vi "FlatToRichcif_can_writer_nixnet_GetCANStatusResponse.vi"(5 "OutputClusterType":T1, 11 "InputCluster":T4) -> (3 "OutputCluster":T1)   [LabVIEW 2021, in "CanWriterNixnet_client.lvlib"]
uses:
  CanWriterNixnet_client.lvlib
  cif_can_writer_nixnet_GetCANStatusResponse_Flat.ctl
  cif_can_writer_nixnet_CommState.ctl
  cif_can_writer_nixnet_LastError.ctl
  cif_can_writer_nixnet_GetCANStatusResponse.ctl
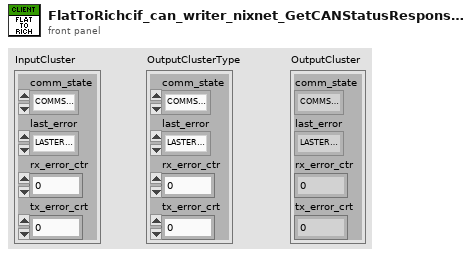
[diagram p1: front panel]
types:
  T1 = typedef "CanWriterNixnet_client.lvlib/cif_can_writer_nixnet_GetCANStatusResponse.ctl" = cluster{"comm_state":T2, "last_error":T3, "rx_error_ctr":u32, "tx_error_crt":u32}
  T2 = typedef "CanWriterNixnet_client.lvlib/cif_can_writer_nixnet_CommState.ctl" = enum32{"COMMSTATE_ERROR_ACTIVE", "COMMSTATE_ERROR_PASSIVE", "COMMSTATE_BUS_OFF"}
  T3 = typedef "CanWriterNixnet_client.lvlib/cif_can_writer_nixnet_LastError.ctl" = enum32{"LASTERROR_NONE", "LASTERROR_STUFF", "LASTERROR_FORM", "LASTERROR_ACK", "LASTERROR_BIT1", "LASTERROR_BIT0", "LASTERROR_CRC", "LASTERROR_UNKNOWN"}
  T4 = typedef "CanWriterNixnet_client.lvlib/cif_can_writer_nixnet_GetCANStatusResponse_Flat.ctl" = cluster{"comm_state":T2, "last_error":T3, "rx_error_ctr":u32, "tx_error_crt":u32}
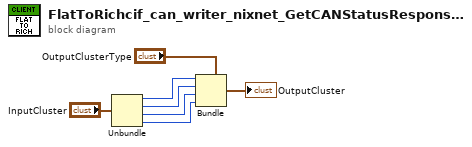
[diagram p0: block diagram]
diagram:
  n1 = Unbundle "Unbundle"("InputCluster") -> ("comm_state"=w4:T2, "last_error"=w3:T3, "rx_error_ctr"=w2:u32, "tx_error_crt"=w1:u32)
  n2 = Bundle "Bundle"(cluster="OutputClusterType", "comm_state"=w4, "last_error"=w3, "rx_error_ctr"=w2, "tx_error_crt"=w1) -> (→"OutputCluster":T1)
